vi "Scanstart error logic.vi"(10 "errors boolean now":bool[](array[boolean]), 11 "scacnstart errors boolean shift reg":bool[](array[boolean])) -> (3 "false is good":bool[](array[boolean]))   [LabVIEW 2020]
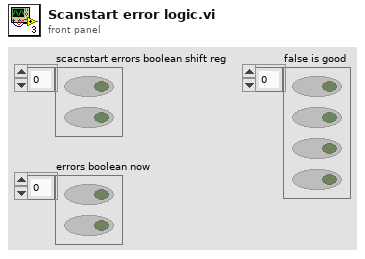
[diagram p1: front panel]
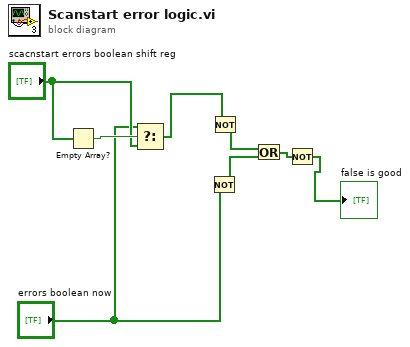
[diagram p0: block diagram]
diagram:
  n1 = Empty Array?(array="scacnstart errors boolean shift reg") -> (empty?=w4:bool)
  n2 = Select(t="errors boolean now", s=w4, f="scacnstart errors boolean shift reg") -> (s? t:f=w1:bool[])
  n3 = Not(x="errors boolean now") -> (.not. x?=w6:bool[])
  n4 = Not(x=w1) -> (.not. x?=w5:bool[])
  n5 = Or(x=w5, y=w6) -> (x .or. y?=w7:bool[])
  n6 = Not(x=w7) -> (.not. x?=→"false is good":bool[])
